vi "CIF Receive Raw.vi"(8 "error in (no error)":errorcluster, 9 "Timeout ms":u32, 10 "Data In":u8[](array[numeric]), 11 "Subscriber Reference":T2 {"refnum" format="%.0x"}) -> (0 "error out":errorcluster, 1 "Array Length":u32, 2 "Data Out":u8[](array[numeric]), 4 "Timeout":bool, 5 "CIF Subscriber Stats":T1)   [LabVIEW 2021, in "Iceoryx.lvlib"]
doc: "Read from an iceoryx CIF pcap queue and read including the flattened CIF header. This is normally used if the payload is being passed as a \"black box\" message such as a TCP stream from another machine. \n\n<B>Data In:</B> Memory location to accept the flattened PCAP formatted data. \n<B>Data Out:</B> The flattened CIF header and the flattened PCAP formatted data. \n<B>Array Length:</B> The length of valid bytes that were copied into the Data Out buffer."
uses:
  Iceoryx.lvlib
  Refnum/Typedef/CIF Subscriber Refnum.ctl
  typedef/CIF Pcap Subscriber Stats.ctl
  SubVIs/Convert Error Core.vi
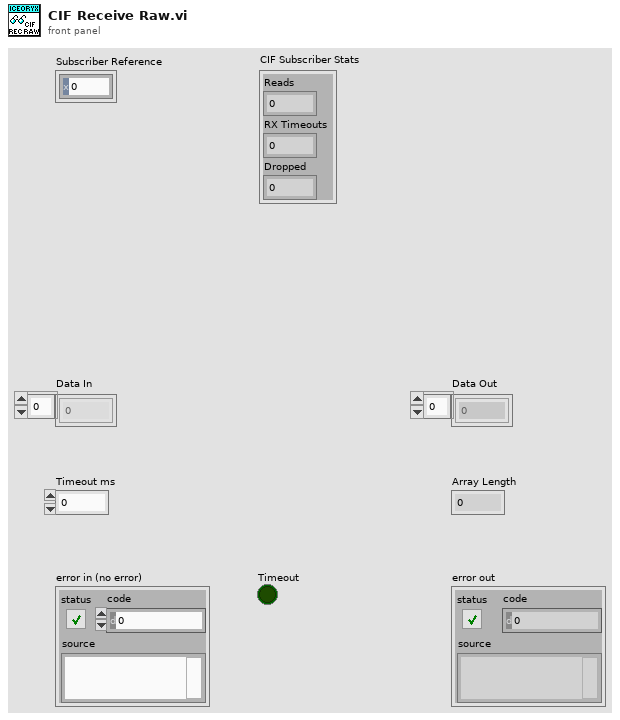
[diagram p1: front panel]
types:
  T1 = typedef "Iceoryx.lvlib/CIF Pcap Subscriber Stats.ctl" = cluster{"Reads":u64, "RX Timeouts":u64, "Dropped":u64}
  T2 = typedef "Iceoryx.lvlib/CIF Subscriber Refnum.ctl" = cluster{"refnum":u64, "CIF Sub":enum8{"cifsub"}}
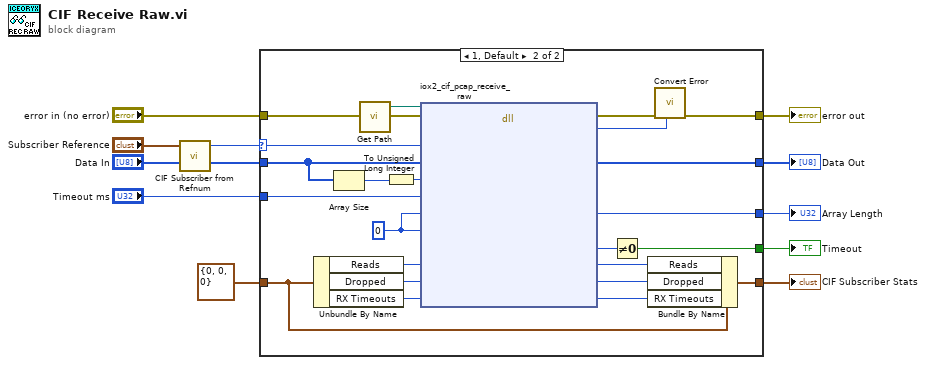
[diagram p0: block diagram]
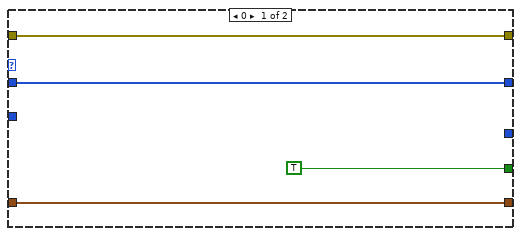
[diagram p2: hidden frame]
diagram:
  n1 = call "CIF Subscriber from Refnum.vi"("CIF Subscriber Refnum"="Subscriber Reference") -> ("CIF Subscriber U64"=w1:u64)  [unwired: 4 in]
  n2 = case shown="1, Default" w1 {
    selector: w1 -> [_ w31]
    tunnel: "error in (no error)" -> [w15 w38]
    tunnel: "Data In" -> [w14 w26]
    tunnel: [w14 w36] -> w4
    tunnel: [w15 w32] -> w10
    tunnel: [_ w30] -> w8
    tunnel: "Timeout ms" -> [_ w29]
    tunnel: [TRUE w27] -> w6
    tunnel: T1 {"Reads"=0, "RX Timeouts"=0, "Dropped"=0} ("CIF Subscriber Stats") -> [w12 w21]
    tunnel: [w12 w17] -> w2
    frame 0 {
    }
    frame 1, Default {
      w37 = u32 0 ("actual")
      n3 = Unbundle By Name(w21) -> ("Reads"=w24:u64, "Dropped"=w22:u64, "RX Timeouts"=w23:u64)
      n4 = Array Size(array=w26) -> (size(s)=w25:i32)
      n5 = call "Get Path.vi"() -> ("libiox2_cif path"=w35:path)  [unwired: 4 in]
      n6 = To Unsigned Long Integer(number=w25) -> (unsigned 32bit integer=w16:u32)
      n7 = dll-call lib="D:/dev/iceoryx2_lvwrapper/dist/iox2_cif.dll" fn="iox2_cif_pcap_receive_raw"(path in=w35, error in=w38, "subscriber"=w31, "sample"=w26, "cap"=w16, "timeout"=w29, "actual"=w37, "max"=w37, "samples"=w24, "dropped"=w22, "timeouts"=w23) -> (error out=w34:errorcluster, "return type"=w33:i32, "sample"=w36:u8[], "actual"=w30:u32, "timed_out"=w28:i32, "samples"=w20:u64, "dropped"=w18:u64, "timeouts"=w19:u64)  [unwired: 6 in, 1 out]
      n8 = Not Equal To 0?(x=w28) -> (x != 0?=w27:bool)
      n9 = Bundle By Name(cluster=w21, "Reads"=w20, "Dropped"=w18, "RX Timeouts"=w19) -> (w17:T1)
      n10 = call "Convert Error.vi"("return type"=w33, "error in (no error)"=w34) -> ("error out"=w32:errorcluster)  [unwired: 9 in]
    }
  }
  "error out" <- w10
  "Array Length" <- w8
  "Timeout" <- w6
  "Data Out" <- w4
  "CIF Subscriber Stats" <- w2
